vi "Channel Estimation.vi"(10 "Half of LLTF":cdb[](array[numeric]), 11 "Frame after fine freq sync in":cdb[](array[numeric])) -> (2 "Channel Estimate":cdb[](array[numeric]))   [LabVIEW 2023]
uses:
  <vilib>/Analysis/NI_AALPro.lvlib
  <vilib>/Analysis/2dsp.llb/Complex FFT.vi
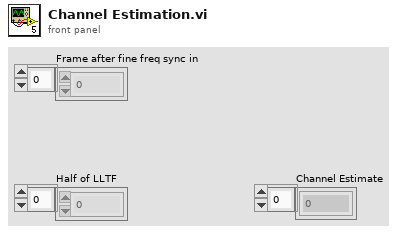
[diagram p1: front panel]
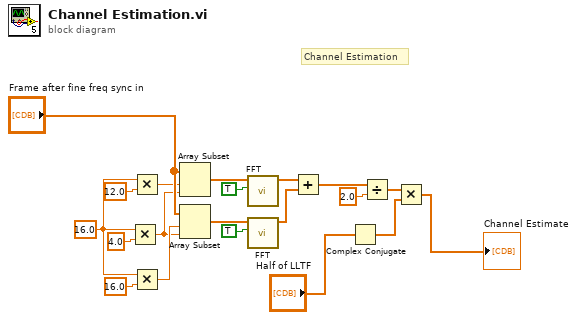
[diagram p0: block diagram]
diagram:
  w1 = 16.0 ("x")
  # "Channel Estimation"
  n1 = Multiply(x=w1, y=4.0) -> (x*y=w6:dbl)
  n2 = Multiply(x=w1, y=12.0) -> (x*y=w5:dbl)
  n3 = Multiply(x=w1, y=16.0) -> (x*y=w7:dbl)
  n4 = Array Subset(array="Frame after fine freq sync in", index=w5, length=w6) -> (w9:cdb[])
  n5 = Array Subset(array="Frame after fine freq sync in", index=w7, length=w6) -> (w8:cdb[])
  n6 = call-poly <vilib>:"FFT.vi"("shift?"=TRUE, "X"=w9) -> ("FFT {X}"=w12:cdb[])  [unwired: 8 in, 1 out]
  n7 = call-poly <vilib>:"FFT.vi"("shift?"=TRUE, "X"=w8) -> ("FFT {X}"=w13:cdb[])  [unwired: 8 in, 1 out]
  n8 = Add(x=w12, y=w13) -> (x+y=w10:cdb[])
  n9 = Complex Conjugate(1:"Half of LLTF") -> (0:w16:cdb[])
  n10 = Divide(x=w10, y=2.0) -> (x/y=w17:cdb[])
  n11 = Multiply(x=w17, y=w16) -> (x*y=→"Channel Estimate":cdb[])
